vi "RemoteVI Remote Target.vi"(0 "put?":bool, 1 "hWnd":u64, 2 "hooks":refnum<vi>, 3 "VI name":string, 5 "remove?":bool) -> (4 "found?":bool, 6 "hooks out":refnum<vi>, 7 "VI name out":string)   [LabVIEW 2020, in "RemoteVI.lvlib"]
doc: "The shares that reach their window's LabVIEW over VI Server (the VI Server route, docs\\architecture.md, Window targets) - a functional global (a Feedback Node outside any loop, initialized on the first call only), keyed by the shared window's hWnd. put? TRUE stores hooks (RemoteVI Remote Hooks.vi opened in that LabVIEW, RemoteVI Connect VI Server.vi) and VI name (the shared VI's name there) for hWnd, replacing an earlier entry; remove? TRUE forgets hWnd; otherwise the entry of hWnd is looked up. found? tells whether hWnd had an entry before this call; hooks out and VI name out are its values. RemoteVI Write Modifiers.vi and RemoteVI Read Panel Info.vi ask it which way to go; the server loop puts the entry after connecting and removes it when it ends."
uses:
  RemoteVI.lvlib
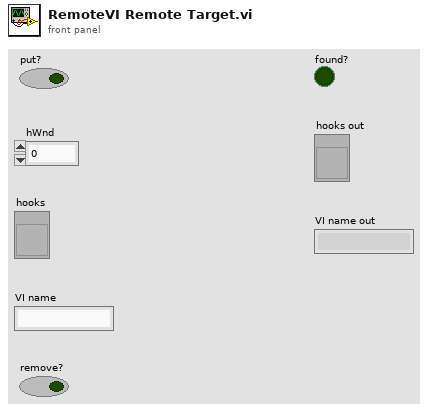
[diagram p1: front panel]
types:
  T1 = cluster{"hWnds":u64[], "hooks":refnum<vi>[], "names":string[]}
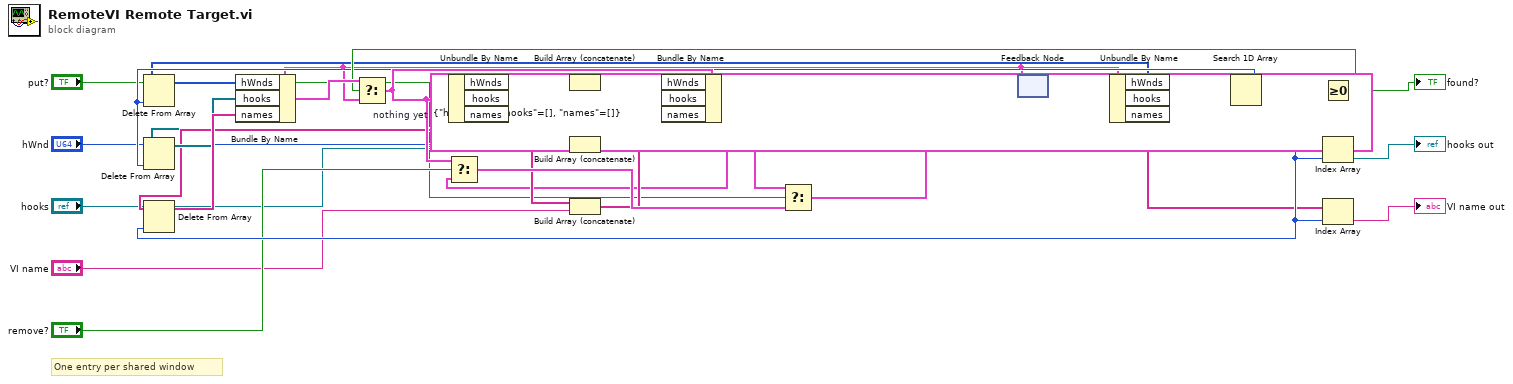
[diagram p0: block diagram]
diagram:
  w6 = T1 {"hWnds"=[], "hooks"=[], "names"=[]}  # nothing yet
  # "One entry per shared window"
  n1 = feedback #1(w6) -> (w7:T1)
  n2 = Unbundle By Name(w7) -> ("hWnds"=w9:u64[], "hooks"=w10:refnum<vi>[], "names"=w11:string[])
  n3 = Search 1D Array(1D array=w9, element="hWnd") -> (index of element=w12:i32)  [unwired: 1 in]
  n4 = Delete From Array(array=w9, index=w12) -> (array with subset deleted=w16:u64[])  [unwired: 1 in, 1 out]
  n5 = Delete From Array(array=w10, index=w12) -> (array with subset deleted=w17:refnum<vi>[])  [unwired: 1 in, 1 out]
  n6 = Delete From Array(array=w11, index=w12) -> (array with subset deleted=w18:string[])  [unwired: 1 in, 1 out]
  n7 = Bundle By Name(cluster=w7, "hWnds"=w16, "hooks"=w17, "names"=w18) -> (w19:T1)
  n8 = Greater Or Equal To 0?(x=w12) -> (x >= 0?=w13:bool)
  "found?" <- w13
  n9 = Select(t=w19, s=w13, f=w7) -> (s? t:f=w20:T1)
  n10 = Unbundle By Name(w20) -> ("hWnds"=w21:u64[], "hooks"=w22:refnum<vi>[], "names"=w23:string[])
  n11 = Select(t=w20, s="remove?", f=w7) -> (s? t:f=w28:T1)
  n12 = Build Array (concatenate)(w21, "hWnd") -> (w24:u64[])
  n13 = Build Array (concatenate)(w22, "hooks") -> (w25:refnum<vi>[])
  n14 = Build Array (concatenate)(w23, "VI name") -> (w26:string[])
  n15 = Bundle By Name(cluster=w20, "hWnds"=w24, "hooks"=w25, "names"=w26) -> (w27:T1)
  n16 = Select(t=w27, s="put?", f=w28) -> (s? t:f=w8:T1)
  n17 = feedback-in #1(w8) -> ()
  n18 = Index Array(array=w10, index=w12) -> (element=→"hooks out":refnum<vi>)
  n19 = Index Array(array=w11, index=w12) -> (element=→"VI name out":string)
